vi "RFH-verify-water_calib_file.vi"(5 "Converted File":path, 7 "Water filepath":path, 8 "error in (no error)":errorcluster, 9 "Max Frequency (6G)":dbl=6000000000.0, 10 "Min Frequency  (0.3G)":dbl=300000000.0) -> (0 "error out":errorcluster, 2 "All Good?":bool, 4 "Converted":T1, 6 "Original":T1)   [LabVIEW 2020, in "RFH-Reflection_File_Handler.lvlib"]
doc: "Verifies a converted water calibration file against the original water file, value by value and in the min and max frequency range. Returns both data sets and whether all is good."
uses:
  RFH-Reflection_File_Handler.lvlib
  RFH-common_data_format_element.ctl
  RFH-common_data_format.ctl
panel:
  out "Range Good?":bool
  out "Values Good?":bool
  out "value 4":T2
  out "value 3":T2
  out "value 2":T2
  out "value":T2
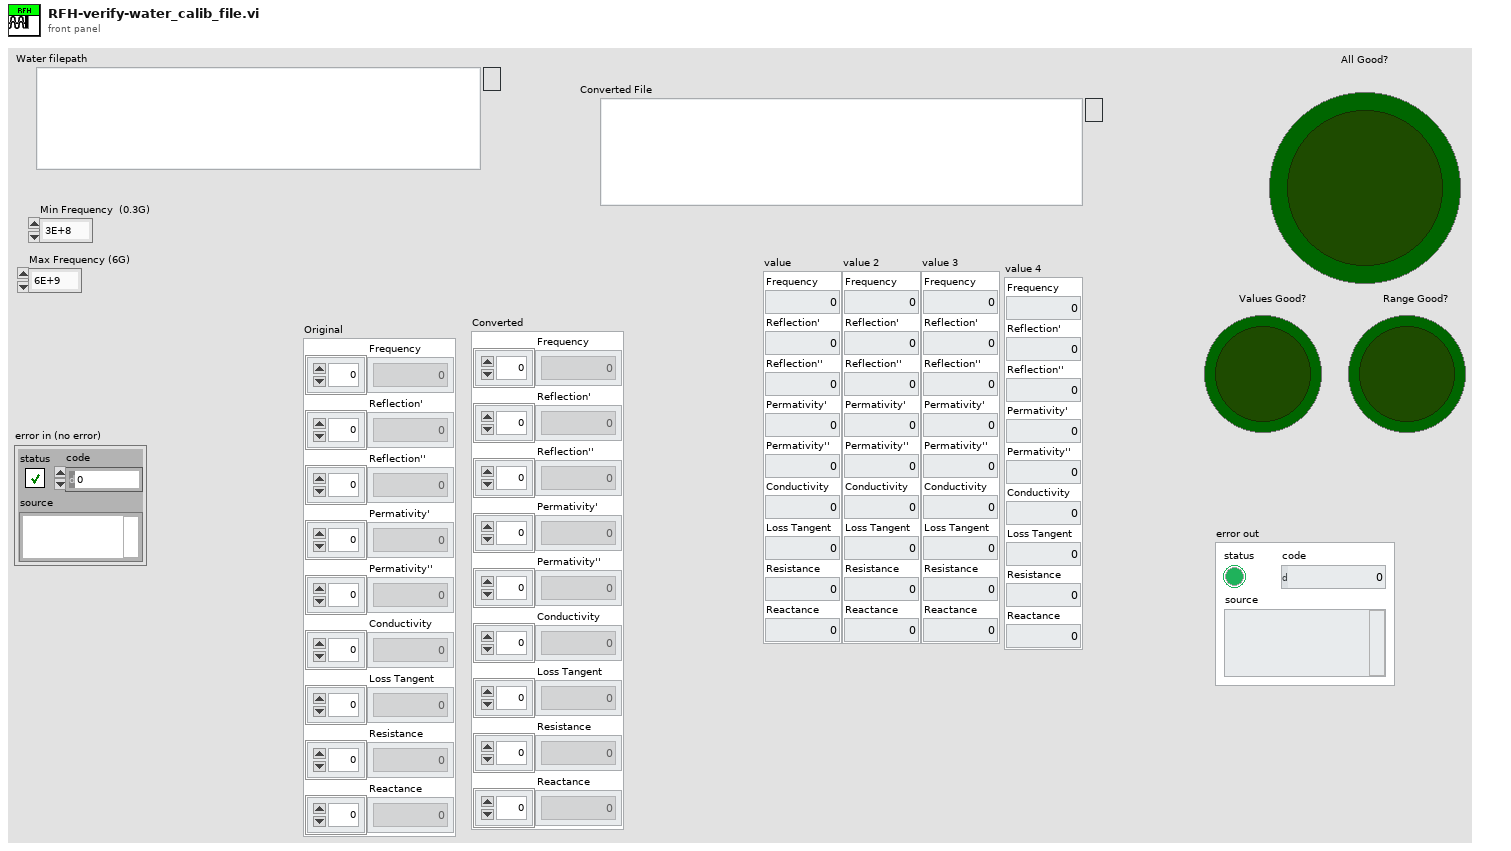
[diagram p1: front panel]
types:
  T1 = typedef "RFH-Reflection_File_Handler.lvlib/RFH-common_data_format.ctl" = cluster{"Frequency":dbl[], "Reflection'":dbl[], "Reflection''":dbl[], "Permativity'":dbl[], "Permativity''":dbl[], "Conductivity":dbl[], "Loss Tangent":dbl[], "Resistance":dbl[], "Reactance":dbl[]}
  T2 = typedef "RFH-Reflection_File_Handler.lvlib/RFH-common_data_format_element.ctl" = cluster{"Frequency":dbl, "Reflection'":dbl, "Reflection''":dbl, "Permativity'":dbl, "Permativity''":dbl, "Conductivity":dbl, "Loss Tangent":dbl, "Resistance":dbl, "Reactance":dbl}
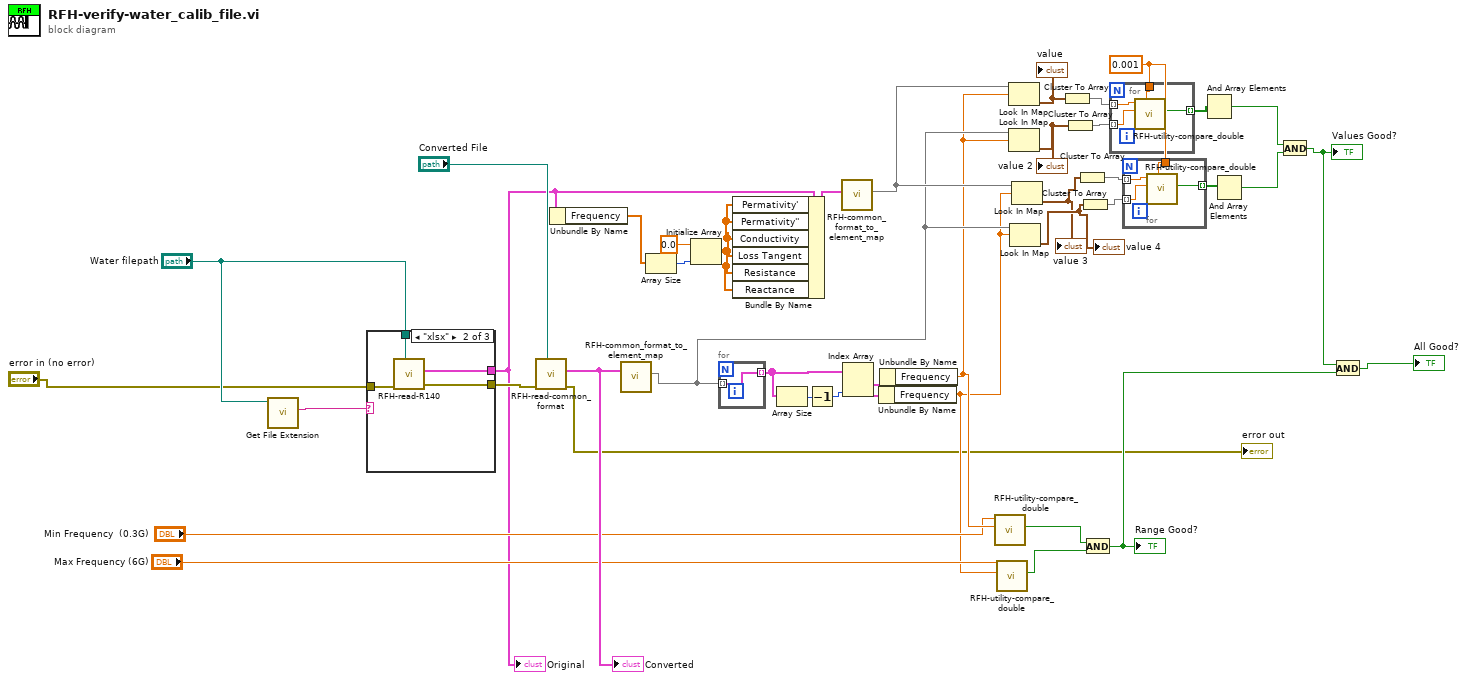
[diagram p0: block diagram]
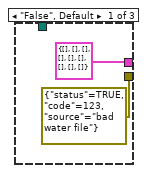
[diagram p2: hidden frame]
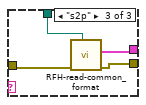
[diagram p3: hidden frame]
diagram:
  w22 = 0.001 ("% tolerance (0.1)")
  n1 = call <vilib>:"Get File Extension.vi"("file"="Water filepath") -> ("lowercase file extension"=w41:string)  [unwired: 6 in, 4 out]
  n2 = case shown="\"xlsx\"" w41 {
    tunnel: [T1 {"Frequency"=[], "Reflection'"=[], "Reflection''"=[], "Permativity'"=[], "Permativity''"=[], "Conductivity"=[], "Loss Tangent"=[], "Resistance"=[], "Reactance"=[]} ("Common Format") w48 w51] -> w1
    tunnel: "Water filepath" -> [_ w47 w52]
    tunnel: [errorcluster {"status"=TRUE, "code"=123, "source"="bad water file"} ("error out") w46 w50] -> w39
    tunnel: "error in (no error)" -> [_ w45 w49]
    frame "False", Default {
    }
    frame "xlsx" {
      n3 = call "RFH-read-R140.vi"("file path (dialog if empty)"=w47, "error in (no error)"=w45) -> ("error out"=w46:errorcluster, "Common Format"=w48:T1)  [unwired: 7 in, 1 out]
    }
    frame "s2p" {
      n4 = call "RFH-read-common_format.vi"("file path (dialog if empty)"=w52, "error in"=w49) -> ("error out"=w50:errorcluster, "Common Format"=w51:T1)  [unwired: 8 in]
    }
  }
  "Original" <- w1
  n5 = call "RFH-read-common_format.vi"("file path (dialog if empty)"="Converted File", "error in"=w39) -> ("error out"=→"error out":errorcluster, "Common Format"=w38:T1)  [unwired: 8 in]
  "Converted" <- w38
  n6 = Unbundle By Name(w1) -> ("Frequency"=w16:dbl[])
  n7 = call "RFH-common_format_to_element_map.vi"("Common Format"=w38) -> ("Element map"=w20:map{dbl, T2})  [unwired: 10 in]
  n8 = Array Size(array=w16) -> (size(s)=w18:i32)
  n9 = Initialize Array(0.0 ("element"), w18) -> (w15:dbl[])
  n10 = for {
    tunnel: w20 -> [w53] mode=indexing
    tunnel: [w53] -> w35 mode=indexing
  }
  n11 = Bundle By Name(cluster=w1, "Permativity'"=w15, "Permativity''"=w15, "Conductivity"=w15, "Loss Tangent"=w15, "Resistance"=w15, "Reactance"=w15) -> (w19:T1)
  n12 = Array Size(array=w35) -> (size(s)=w36:i32)
  n13 = Decrement(x=w36) -> (x-1=w37:i32)
  n14 = call "RFH-common_format_to_element_map.vi"("Common Format"=w19) -> ("Element map"=w21:map{dbl, T2})  [unwired: 10 in]
  n15 = Index Array(array=w35, index #2=w37) -> (element #1=w33:cluster{"Frequency":dbl, "Common Format":T2}, element #2=w34:cluster{"Frequency":dbl, "Common Format":T2})  [unwired: 1 in]
  n16 = Unbundle By Name(w34) -> ("Frequency"=w9:dbl)
  n17 = Unbundle By Name(w33) -> ("Frequency"=w12:dbl)
  n18 = call "RFH-utility-compare_double.vi"("New"=w12, "original"="Min Frequency  (0.3G)") -> ("In Range?"=w8:bool)  [unwired: 9 in]
  n19 = call "RFH-utility-compare_double.vi"("New"=w9, "original"="Max Frequency (6G)") -> ("In Range?"=w7:bool)  [unwired: 9 in]
  n20 = Look In Map(map=w21, key=w12) -> (value=w32:T2)  [unwired: 1 in, 1 out]
  "value" <- w32
  n21 = Look In Map(map=w20, key=w12) -> (value=w31:T2)  [unwired: 1 in, 1 out]
  "value 2" <- w31
  n22 = Look In Map(map=w20, key=w9) -> (value=w26:T2)  [unwired: 1 in, 1 out]
  "value 4" <- w26
  n23 = Look In Map(map=w21, key=w9) -> (value=w25:T2)  [unwired: 1 in, 1 out]
  "value 3" <- w25
  n24 = Cluster To Array(cluster=w32) -> (array=w30:dbl[])
  n25 = Cluster To Array(cluster=w31) -> (array=w29:dbl[])
  n26 = Cluster To Array(cluster=w25) -> (array=w27:dbl[])
  n27 = Cluster To Array(cluster=w26) -> (array=w28:dbl[])
  n28 = And(x=w8, y=w7) -> (x .and. y?=w6:bool)
  "Range Good?" <- w6
  n29 = for {
    tunnel: w30 -> [w57] mode=indexing
    tunnel: w29 -> [w56] mode=indexing
    tunnel: [w55] -> w23 mode=indexing
    tunnel: w22 -> [w54]
    n30 = call "RFH-utility-compare_double.vi"("% tolerance (0.1)"=w54, "New"=w56, "original"=w57) -> ("In Range?"=w55:bool)  [unwired: 8 in]
  }
  n31 = for {
    tunnel: w27 -> [w61] mode=indexing
    tunnel: w28 -> [w60] mode=indexing
    tunnel: [w59] -> w24 mode=indexing
    tunnel: w22 -> [w58]
    n32 = call "RFH-utility-compare_double.vi"("% tolerance (0.1)"=w58, "New"=w60, "original"=w61) -> ("In Range?"=w59:bool)  [unwired: 8 in]
  }
  n33 = And Array Elements(Boolean array=w23) -> (logical AND=w14:bool)
  n34 = And Array Elements(Boolean array=w24) -> (logical AND=w13:bool)
  n35 = And(x=w14, y=w13) -> (x .and. y?=w3:bool)
  "Values Good?" <- w3
  n36 = And(x=w3, y=w6) -> (x .and. y?=→"All Good?":bool)
